vi "Main.vi"(11 "Module Admin":refnum<class "Delacor_lib_QMH_Module Admin.lvclass">) -> ()   [LabVIEW 2026, in "Replay.lvlib"]
doc: "This template is based off of the Queued Message Handler design pattern and the Queued Message Handler project template that ships with LabVIEW.\n\nThe main difference is that the queue is private to this module and communication between modules is performed via Broadcast and Request events.\n\nRequest events are wrapped in public API methods and are handled in the Event Handling Loop (EHL) of this VI. Any module can register for Broadcast events sent by this module. The EHL generates messages based on user interface actions.\n\nThe Message Handling Loop (MHL) processes messages generated by the EHL, or by other messages. The messages are string values, so new messages can be added easily to the Message Cases case structure in the MHL. Each message cluster can also provide an optional value for Message Data, which is a variant that can be converted to whatever message-specific data is required.\n_____\nBased on DQMH Dev Tools: Project Template 7.1.2.1547."
uses:
  Replay.lvlib
  <vilib>/Delacor/Delacor QMH/Libraries/Module Admin_class/Delacor_lib_QMH_Module Admin.lvclass
  <vilib>/Wovalab/Utilities/Helper Loop Periodic Timing/Late Execution Mode--enum.ctl
  <vilib>/Wovalab/Utilities/Helper Loop Periodic Timing/Helper Loop Periodic Timing.lvclass/Helper Loop Periodic Timing.ctl
  Replay MH Loop.ctl
  Replay Helper Loop.ctl
  <vilib>/Delacor/Delacor QMH/Libraries/Message Queue_class/Delacor_lib_QMH_Message Queue.lvclass/Delacor_lib_QMH_Message Queue.ctl
  Stop Argument--cluster.ctl
  <vilib>/Delacor/Delacor QMH/Libraries/Module Admin_class/Delacor_lib_QMH_Module Admin.lvclass/Delacor_lib_QMH_Module Admin.ctl
  Load UserEvents Argument--cluster.ctl
  Load UserEvents (Reply Payload)--cluster.ctl
  <vilib>/Utility/miscctls.llb/LVPointTypeDef.ctl
  modules/coordinator/src/Libraries/UserEventRecorder/KeyboardAndMouseDataAcquisition.ctl
  <vilib>/Delacor/Delacor QMH/Libraries/Message Queue_class/Delacor_lib_QMH_Enqueue Message (Single).vi
  <vilib>/Delacor/Delacor QMH/Libraries/Module Admin_class/Delacor_lib_QMH_Get External Launch.vi
  <vilib>/Wovalab/Utilities/Helper Loop Periodic Timing/Stop Helper Loop.vi
  <vilib>/Wovalab/Utilities/Helper Loop Periodic Timing/Stop Helper Loop Internal.vi
  <vilib>/Wovalab/Utilities/Helper Loop Periodic Timing/U32 Max Value--constant.vi
  <vilib>/Wovalab/Utilities/Helper Loop Periodic Timing/Update Last Execution Time.vi
  <vilib>/Wovalab/Utilities/Helper Loop Periodic Timing/Loops Events AE.vi
  <vilib>/Wovalab/Utilities/Helper Loop Periodic Timing/Notify Monitoring Window.vi
  <vilib>/Wovalab/Utilities/Helper Loop Periodic Timing/Monitoring--global.vi
  <vilib>/Wovalab/Utilities/Helper Loop Periodic Timing/Helper Loop Periodic Timing.lvclass
  <vilib>/Delacor/Delacor QMH/Libraries/Message Queue_class/Delacor_lib_QMH_Message Queue.lvclass
  modules/coordinator/src/Libraries/Launcher/Launcher.lvlib
panel:
  out "Late?":bool
  out "First Execution Since Period Modification?":bool
  out "error out":errorcluster
  out "Status":string
  in  "Simulate MHL Error":bool
  in  "Simulate EHL Error":bool
  # "Other processes communicate with this Module via its Public API (wrappers for its Request Events).\n\nThis Module communicates with other processes via its Broadcast Events.\nAny process that wants to receive these messages can register for this module's Broadcast events."
  # "This template is for the DQMH framework. See the block diagram for more information on how to use this template."
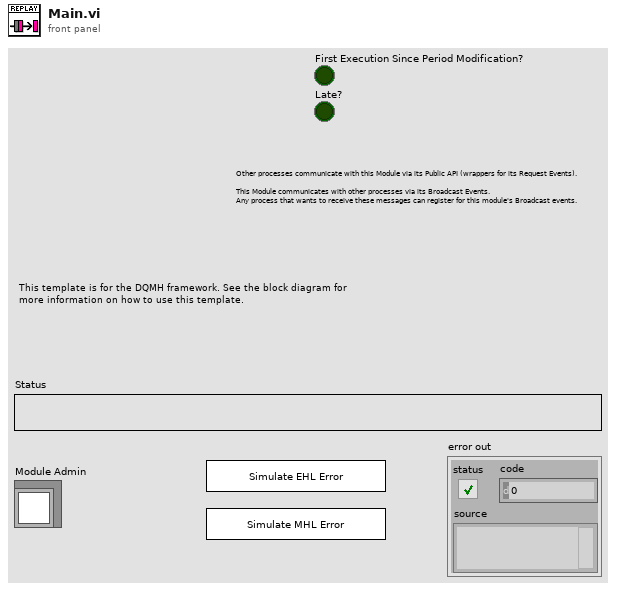
[diagram p1: front panel]
types:
  T1 = typedef "Wovalab_lib_Utilities.lvlib/Helper Loop Periodic Timing.lvclass/Late Execution Mode--enum.ctl" = enum16{"No change", "Process missed periods ignoring original phase", "Process missed periods maintaining original phase"}
  T2 = typedef "Replay.lvlib/Request Events--cluster.ctl" = cluster{"Stop Module":refnum<user-event>, "Show Panel":refnum<user-event>, "Hide Panel":refnum<user-event>, "Get Module Execution Status":refnum<user-event>, "Show Diagram":refnum<user-event>, "Set Run ID to Replay":refnum<user-event>, "Load UserEvents":refnum<user-event>, "Private.Trigger Replay Metadata":refnum<user-event>}
  T3 = typedef "Launcher.lvlib/Broadcast Events--cluster.ctl" = cluster{"Module Did Init":refnum<user-event>, "Status Updated":refnum<user-event>, "Error Reported":refnum<user-event>, "Module Did Stop":refnum<user-event>, "Update Module Execution Status":refnum<user-event>, "Start Capture Detection Loop":refnum<user-event>, "Benchmark Started":refnum<user-event>, "Broadcast number of frames and run ID":refnum<user-event>}
  T4 = typedef "Replay.lvlib/Replay Helper Loop.ctl" = cluster{"Run ID":string, "Sample Number":i32, "Load From Program Data":bool}
  T5 = typedef "Replay.lvlib/Replay MH Loop.ctl" = cluster{"Run ID":string, "Frame Index":i32}
  T6 = enum32{"invalid lock state", "Not Locked", "Locked (No Password)", "Password-protected"}
  T7 = typedef "Replay.lvlib/Stop Argument--cluster.ctl" = cluster{"Origin":string, "Exit via Stop Module Req?":bool, "Wait for Module to stop?":bool}
  T8 = typedef "Replay.lvlib/Load UserEvents Argument--cluster.ctl" = cluster{"Run ID":string, "Wait Notifier":refnum<notifier>, "wait for reply":bool, "Load From Program Data":bool}
  T9 = typedef "LVPointTypeDef.ctl" = cluster{"Horizontal":i16, "Vertical":i16}
  T10 = enum32{"Invalid", "Standard", "Closed", "Hidden", "Minimized", "Maximized"}
  T11 = typedef "Replay.lvlib/Load UserEvents (Reply Payload)--cluster.ctl" = cluster{"error":errorcluster, "Run ID":string, "Load From Program Data":bool}
  T12 = typedef "KeyboardAndMouseDataAcquisition.ctl" = cluster{"axis info":cluster{"Horizontal":i32, "Vertical":i32, "Scrolling":i32}, "button info":cluster{"button 1":bool, "button 2":bool, "button 3":bool, "button 4":bool}, "Relative Time (User Event)":dbl, "Sample Number":u32, "Relative Time (Frame 0)":dbl, "key mode":enum16{"RELATIVE", "ABSOLUTE"}, "Frame Number":u32, "Keyboard Key Pressed":enum16{"0", "1", "2", "3", "4", "5", "6", "7", "8", "9", "A", "B", "C", "D", "E", "F", "G", "H", "I", "J", "K", "L", "M", "N", "O", "P", "Q", "R", "S", "T", "U", "V", "W", "X", "Y", "Z", "F1", "F2", "F3", "F4", "F5", "F6", "F7", "F8", "F9", "F10", "F11", "F12", "F13", "F14", "F15", "ADD", "BACK", "BACKSLASH", "CAPITAL", "COMMA", "DECIMAL", "DELETE", "DIVIDE", "DOWN", "END", "EQUALS", "ESCAPE", "GRAVE (`)", "HOME", "INSERT", "LBRACKET", "LCONTROL", "LEFT", "L ALT", "LSHIFT", "LWIN", "MINUS", "MULTIPLY", "NEXT", "NUMLOCK", "NUMPAD_0", "NUMPAD_1", "NUMPAD_2", "NUMPAD_3", "NUMPAD_4", "NUMPAD_5", "NUMPAD_6", "NUMPAD_7", "NUMPAD_8", "NUMPAD_9", "PAUSE", "PERIOD", "PRIOR (PG UP)", "RBRACKET", "RCONTROL", "RETURN", "RIGHT", "R ALT", "RSHIFT", "RWIN", "SCROLL", "SEMICOLON", "SLASH", "SPACE", "SUBTRACT", "TAB", "UP", "ENTER (num pad)", "' (quote)"}, "Keyboard No Op":bool}
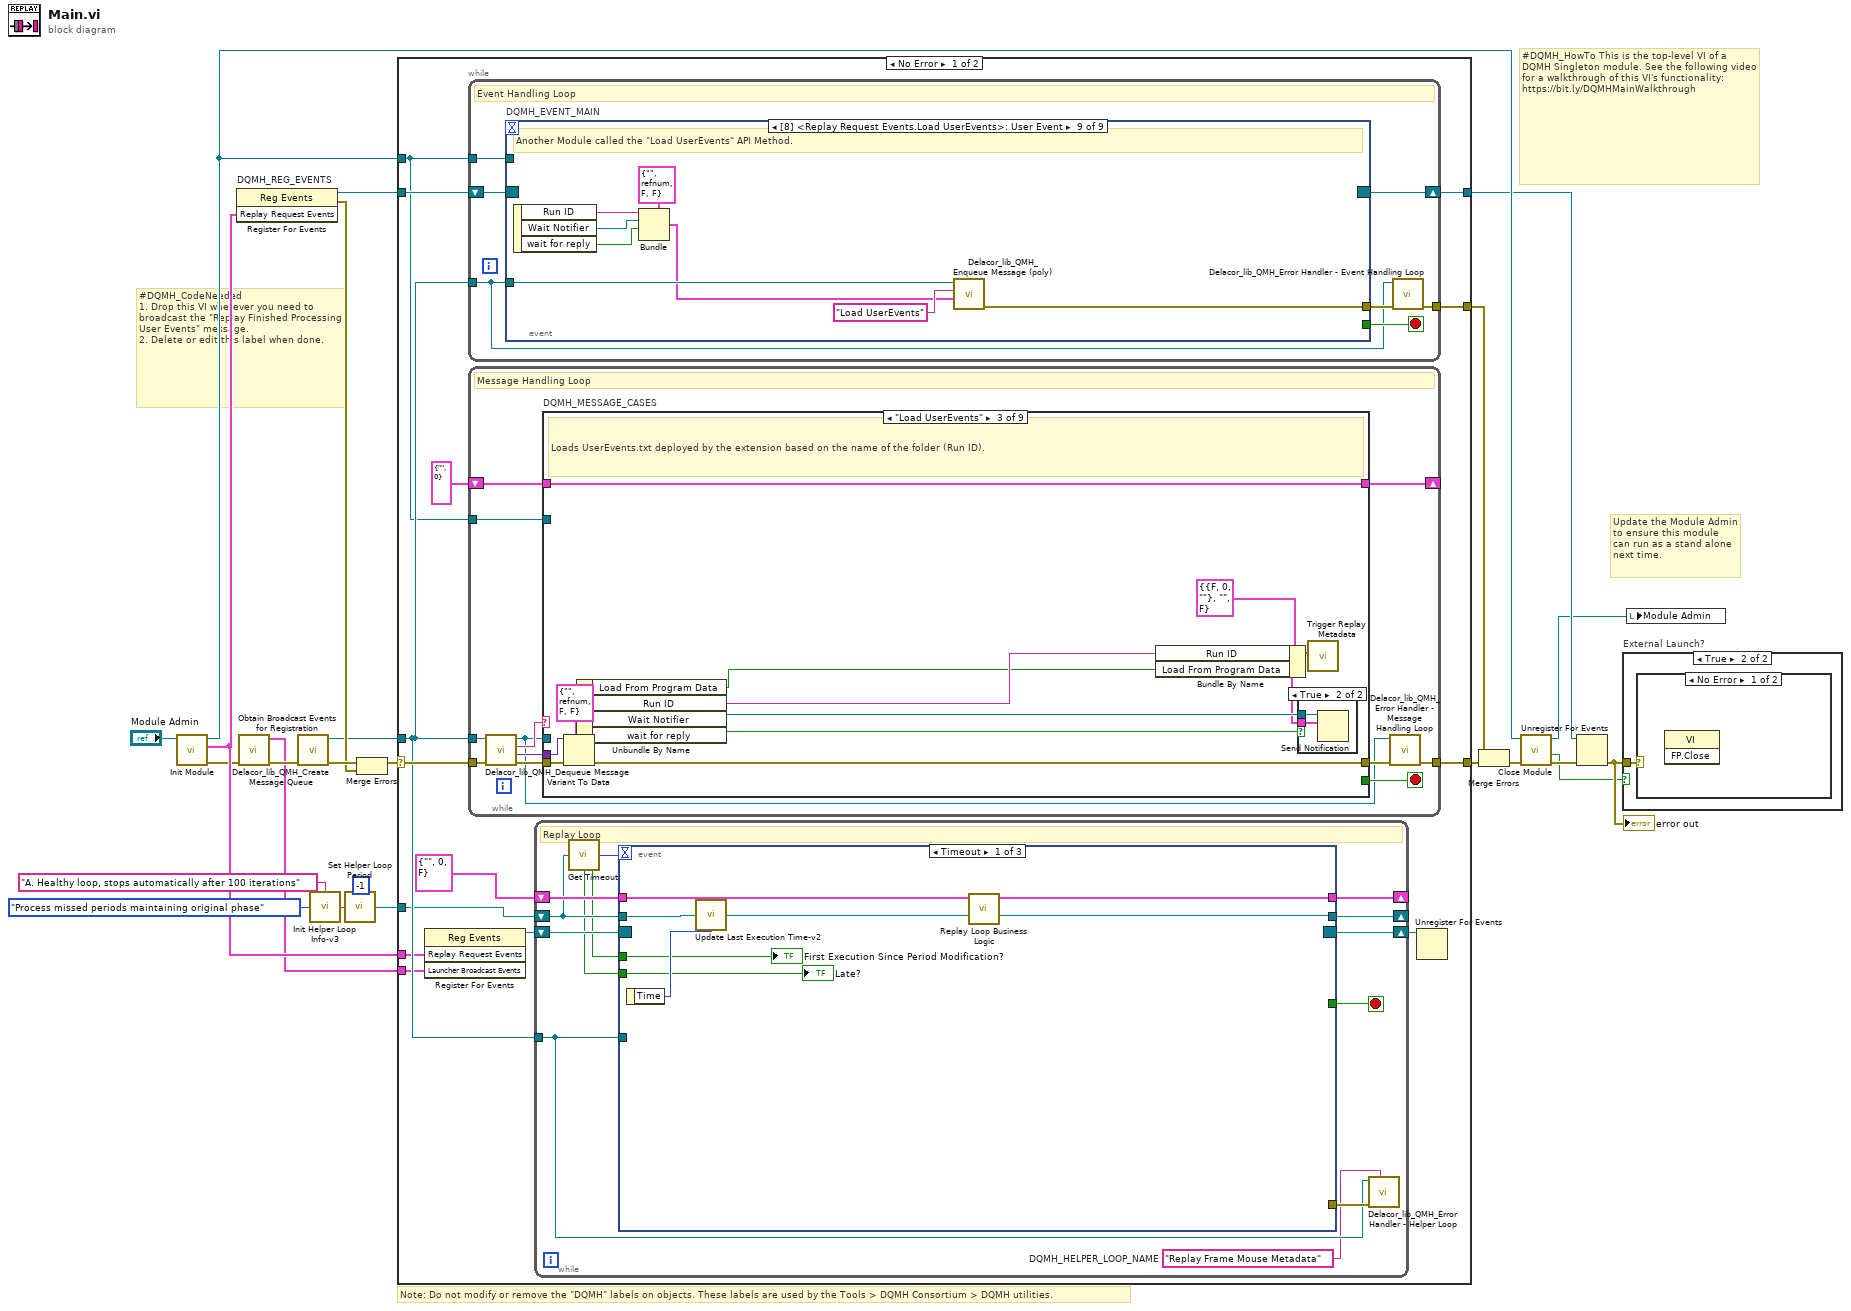
[diagram p0: block diagram]
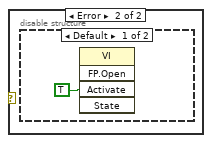
[diagram p3: hidden frame]
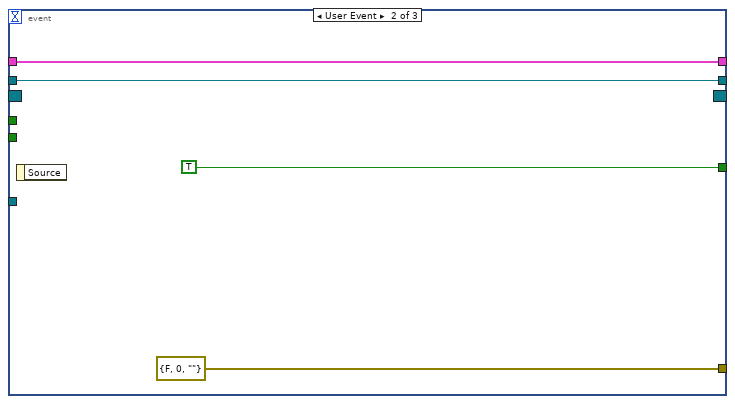
[diagram p5: hidden frame]
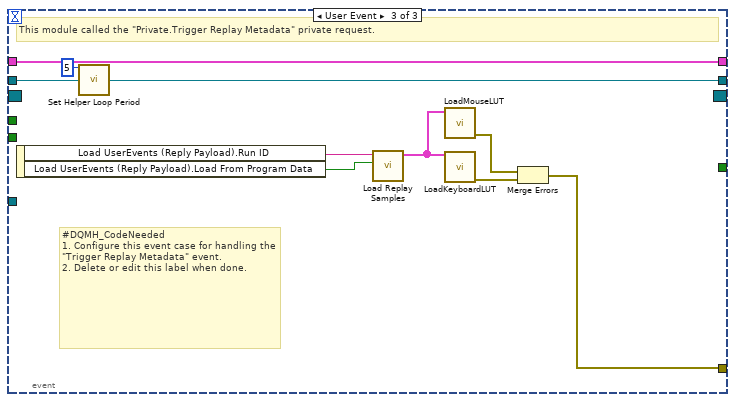
[diagram p6: hidden frame]
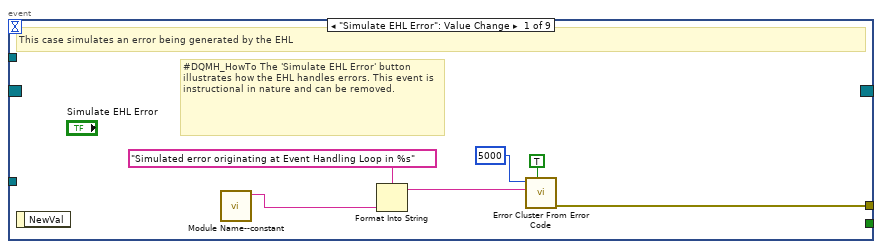
[diagram p7: hidden frame]
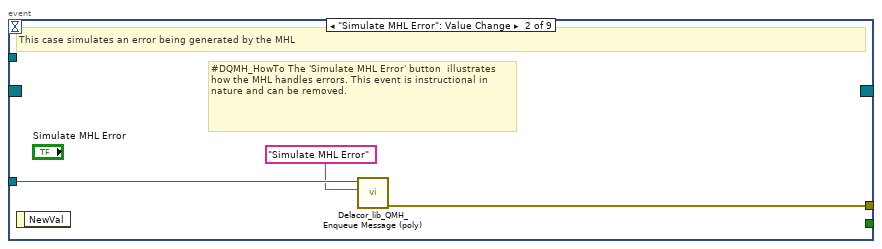
[diagram p8: hidden frame]
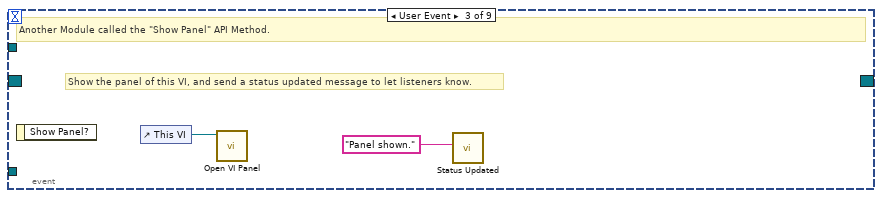
[diagram p9: hidden frame]
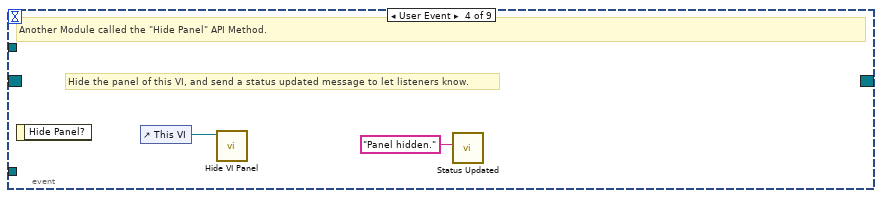
[diagram p10: hidden frame]
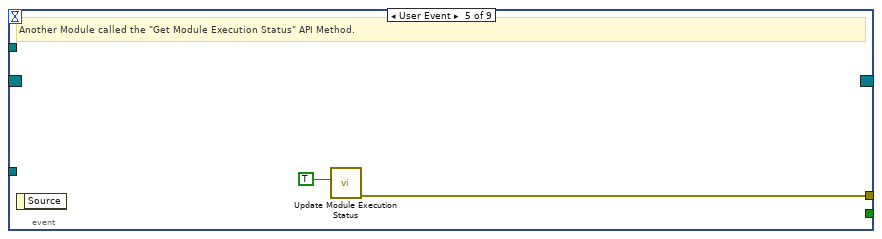
[diagram p11: hidden frame]
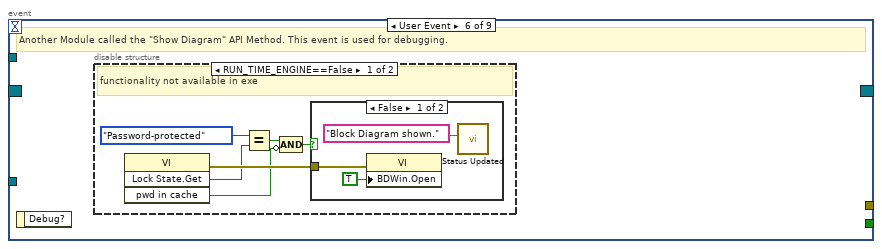
[diagram p12: hidden frame]
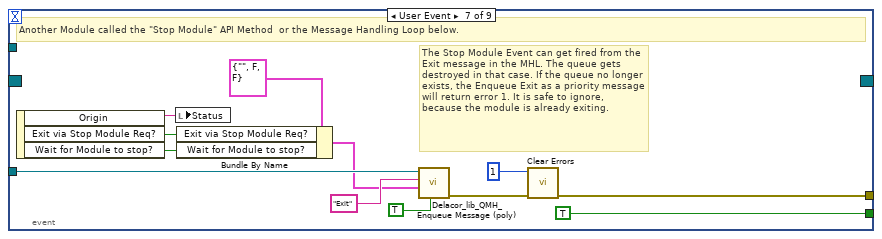
[diagram p15: hidden frame]
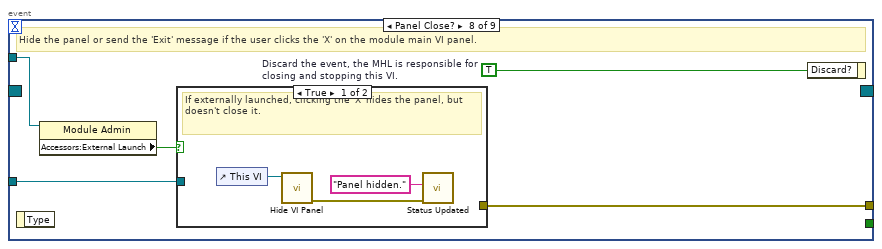
[diagram p16: hidden frame]
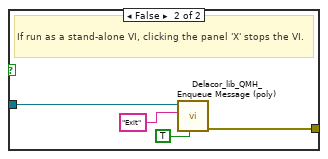
[diagram p17: hidden frame]
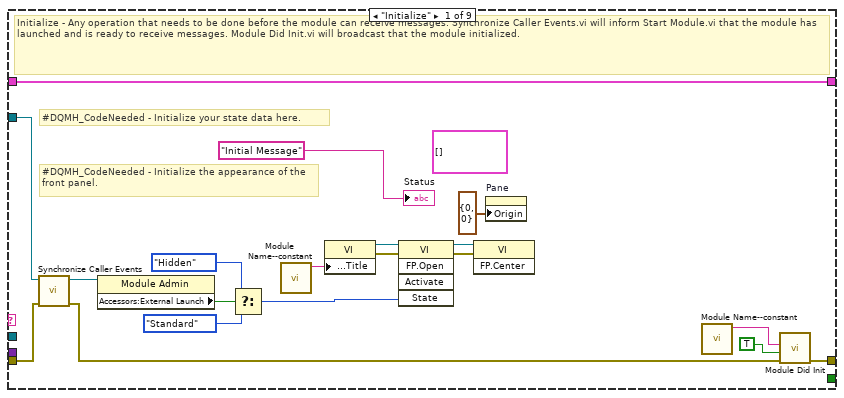
[diagram p18: hidden frame]
diagram:
  # "#DQMH_CodeNeeded\n1. Drop this VI wherever you need to fire the \"Private.Trigger Replay Metadata\" event.\n2. Delete or edit this label when done."
  # "#DQMH_CodeNeeded\n1. Drop this VI wherever you need to broadcast the \"Replay Finished Processing User Events\" message.\n2. Delete or edit this label when done."
  # "#DQMH_HowTo This is the top-level VI of a DQMH Singleton module. See the following video for a walkthrough of this VI's functionality: https://bit.ly/DQMHMainWalkthrough"
  # "Note: Do not modify or remove the \"DQMH\" labels on objects. These labels are used by the Tools > DQMH Consortium > DQMH utilities."
  # "Update the Module Admin to ensure this module can run as a stand alone next time."
  n1 = call "Init Module.vi"("Singleton Module Admin in"="Module Admin") -> ("error out"=w8:errorcluster, "Replay Request Events"=w9:T2, "Singleton Module Admin out"=w16:refnum<class "Delacor_lib_QMH_Module Admin.lvclass">)  [unwired: 8 in]
  n2 = register-events "DQMH_REG_EVENTS"(w9) -> (reference out=w14:refnum<event-registration>, error out=w17:errorcluster)  [unwired: 2 in]
  n3 = call "Obtain Broadcast Events for Registration.vi"("error in"=w8) -> ("error out"=w7:errorcluster, "Launcher Broadcast Events"=w6:T3)  [unwired: 8 in, 1 out]
  n4 = call <vilib>:"Delacor_lib_QMH_Create Message Queue.vi"("error in"=w7) -> ("error out"=w19:errorcluster, "Message Queue"=w13:refnum<class "Delacor_lib_QMH_Message Queue.lvclass">)  [unwired: 9 in]
  n5 = call <vilib>:"Init Helper Loop Info-v3.vi"("Late Execution Mode (Process missed periods ignoring original phase)"=Late_Execution_Mode--enum."Process missed periods maintaining original phase", "Loop Name (\"\": Caller VI)"="A. Healthy loop, stops automatically after 100 iterations" ("Loop Name (\"\": Caller VI)")) -> ("Helper Loop Periodic Timing"=w4:refnum<class "Helper Loop Periodic Timing.lvclass">)
  n6 = call <vilib>:"Set Helper Loop Period.vi"("Period (ms)"=-1, "Helper Loop Periodic Timing in"=w4) -> ("Helper Loop Periodic Timing out"=w2:refnum<class "Helper Loop Periodic Timing.lvclass">)  [unwired: 13 in]
  n7 = Merge Errors(w19, w17) -> (w18:errorcluster)
  n8 = case shown="No Error" w18 {
    selector: w18 -> [w36 w246]
    tunnel: [w38 w245] -> w24
    tunnel: [w35 w244] -> w15
    tunnel: w14 -> [w34 w244]
    tunnel: w13 -> [w33 w239]
    tunnel: [w37 _] -> w22
    tunnel: w16 -> [w32 w240]
    tunnel: w9 -> [w31 _]
    tunnel: w6 -> [w28 _]
    tunnel: w2 -> [w27 _]
    frame No Error {
      n9 = register-events ("DQMH_HELPER_REGFOREVENTS")(w31, w28) -> (reference out=w29:refnum<event-registration>)  [unwired: 2 in, 1 out]
      n10 = while {
        tunnel: w33 -> [w73]
        shift-right: [w76] -> w35
        shift-left: w34 -> [w77]
        tunnel: [w78] -> w37
        tunnel: w32 -> [w74]
        stop <- w75 stop-if-true
        # "Event Handling Loop"
        n11 = event "DQMH_EVENT_MAIN" shown="[8] <Replay Request Events.Load UserEvents>: User Event" {
          selector: w77 -> [_ _ _ _ _ _ _ _ _]
          dyn-events: [_ _ _ _ _ _ _ _ _] -> w76
          timeout: _ -> [_ _ _ _ _ _ _ _ _]
          tunnel: [_ _ _ _ _ _ TRUE ("Discard?") _ _] -> w75
          tunnel: w73 -> [_ w87 _ _ _ _ w111 w118 w135]
          tunnel: [w85 w88 _ _ w94 _ w114 w120 w128] -> w79
          tunnel: w74 -> [_ _ _ _ _ _ _ w117 _]
          event "Simulate EHL Error": Value Change {
            # "#DQMH_HowTo The 'Simulate EHL Error' button  illustrates how the EHL handles errors. This event is instructional in nature and can be removed."
            # "This case simulates an error being generated by the EHL"
            n12 = event-data() -> ()  [unwired: 1 in, 1 out]
            n13 = call "Module Name--constant.vi"() -> ("Module Name"=w82:string)  [unwired: 11 in]
            n14 = Format Into String(format string="Simulated error originating at Event Handling Loop in %s", w82) -> (resulting string=w83:string)  [unwired: 2 in, 1 out]
            n15 = call <vilib>:"Error Cluster From Error Code.vi"("show call chain? (False)"=TRUE, "error message (\"\")"=w83, "error code (0)"=5000) -> ("error out"=w85:errorcluster)  [unwired: 6 in]
          }
          event "Simulate MHL Error": Value Change {
            # "#DQMH_HowTo The 'Simulate MHL Error' button  illustrates how the MHL handles errors. This event is instructional in nature and can be removed."
            # "This case simulates an error being generated by the MHL"
            n16 = event-data() -> ()  [unwired: 1 in, 1 out]
            n17 = call-poly <vilib>:"Delacor_lib_QMH_Enqueue Message (poly).vi"("Message"="Simulate MHL Error", "Message Queue in"=w87) -> ("error out"=w88:errorcluster)  [unwired: 8 in, 1 out]
          }
          event User Event {
            # "Show the panel of this VI, and send a status updated message to let listeners know."
            # "Another Module called the \"Show Panel\" API Method."
            n18 = event-data() -> ()  [unwired: 1 in, 1 out]
            n19 = control-ref of="This VI"() -> (w90:refnum<vi>)
            n20 = call "Open VI Panel.vi"("VI"=w90) -> ()  [unwired: 10 in, 1 out]
            n21 = call "Status Updated.vi"("Status"="Panel shown." ("format string")) -> ()  [unwired: 10 in, 1 out]
          }
          event User Event {
            # "Hide the panel of this VI, and send a status updated message to let listeners know."
            # "Another Module called the \"Hide Panel\" API Method."
            n22 = event-data() -> ()  [unwired: 1 in, 1 out]
            n23 = control-ref of="This VI"() -> (w92:refnum<vi>)
            n24 = call "Hide VI Panel.vi"("VI"=w92) -> ()  [unwired: 10 in, 1 out]
            n25 = call "Status Updated.vi"("Status"="Panel hidden." ("format string")) -> ()  [unwired: 10 in, 1 out]
          }
          event User Event {
            # "Another Module called the \"Get Module Execution Status\" API Method."
            n26 = event-data() -> ()  [unwired: 1 in, 1 out]
            n27 = call "Update Module Execution Status.vi"("Running?"=TRUE) -> ("error out"=w94:errorcluster)  [unwired: 10 in]
          }
          event User Event {
            # "Another Module called the \"Show Diagram\" API Method. This event is used for debugging."
            n28 = event-data() -> ()  [unwired: 1 in, 1 out]
            n29 = disable-structure shown="RUN_TIME_ENGINE==False" {
              frame condition #0 (active) {
                # "functionality not available in exe"
                n30 = invoke on="Invoke Node" class="VI" method="Lock State.Get"() -> (error out=w100:errorcluster, "Get Lock State"=w99:T6, "pwd in cache"=w96:bool)  [unwired: 4 in, 1 out]
                n31 = Equal?(x=T6."Password-protected", y=w99) -> (x = y?=w97:bool)
                n32 = Compound Arithmetic op=AND(w97, invert w96) -> (w95:bool)
                n33 = case shown="False" w95 {
                  tunnel: w100 -> [w103 _]
                  frame False {
                    n34 = property on="Property Node" class="VI"(error in=w103, "BDWin.Open"=TRUE ("Block Diagram Window:Open")) -> ()  [unwired: 1 in, 2 out]
                    n35 = call "Status Updated.vi"("Status"="Block Diagram shown." ("format string")) -> ()  [unwired: 10 in, 1 out]
                  }
                  frame True {
                    # "Password-protected VI, and the password is not in the cache. Do not show the diagram."
                  }
                }
              }
              frame condition #1 {
              }
            }
          }
          event User Event {
            # "The Stop Module Event can get fired from the Exit message in the MHL. The queue gets destroyed in that case. If the queue no longer exists, the Enqueue Exit as a priority message will return error 1. It is safe to ignore, because the module is already exiting."
            # "Another Module called the \"Stop Module\" API Method  or the Message Handling Loop below."
            n36 = event-data() -> ("Origin"=w110:string, "Exit via Stop Module Req?"=w106:bool, "Wait for Module to stop?"=w105:bool)  [unwired: 1 in]
            n37 = local write "Status"(w110) -> ()
            n38 = Bundle By Name(cluster=T7 {"Origin"="", "Exit via Stop Module Req?"=FALSE, "Wait for Module to stop?"=FALSE} ("Stop Argument"), "Exit via Stop Module Req?"=w106, "Wait for Module to stop?"=w105) -> (w104:T7)
            n39 = call-poly <vilib>:"Delacor_lib_QMH_Enqueue Message (poly).vi"("Priority Message? (F)"=TRUE, "Message Data"=w104, "Message"="Exit", "Message Queue in"=w111) -> ("error out"=w115:errorcluster)  [unwired: 6 in, 1 out]
            n40 = call <vilib>:"Clear Errors.vi"("error in (no error)"=w115, "specific error code to clear (0: all)"=1) -> ("error out"=w114:errorcluster)  [unwired: 4 in, 1 out]
          }
          event Panel Close? {
            w119 = TRUE  # Discard the event, the MHL is responsible for closing and stopping this VI.
            # "Hide the panel or send the 'Exit' message if the user clicks the 'X' on the module main VI panel."
            n41 = event-data() -> ()  [unwired: 1 in, 1 out]
            n42 = property on="Property Node" class="Module Admin"(reference=w117) -> ("Accessors:External Launch"=w116:bool)  [unwired: 1 in, 2 out]
            n43 = case shown="True" w116 {
              tunnel: w118 -> [_ w126]
              tunnel: [_ w127] -> w120
              frame True {
                # "If externally launched, clicking the 'X' hides the panel, but doesn't close it."
                n44 = control-ref of="This VI"() -> (w123:refnum<vi>)
                n45 = call "Hide VI Panel.vi"("VI"=w123) -> ("error out"=w121:errorcluster)  [unwired: 10 in]
                n46 = call "Status Updated.vi"("error in"=w121, "Status"="Panel hidden." ("format string")) -> ()  [unwired: 9 in, 1 out]
              }
              frame False {
                # "If run as a stand-alone VI, clicking the panel 'X' stops the VI."
                n47 = call-poly <vilib>:"Delacor_lib_QMH_Enqueue Message (poly).vi"("Priority Message? (F)"=TRUE, "Message"="Exit", "Message Queue in"=w126) -> ("error out"=w127:errorcluster)  [unwired: 7 in, 1 out]
              }
            }
            n48 = event-data ("Event Filter Node")("Discard?"=w119) -> ()  [unwired: 1 in, 1 out]
          }
          event User Event {
            # "Another Module called the \"Load UserEvents\" API Method."
            n49 = event-data() -> ("Run ID"=w131:string, "Wait Notifier"=w130:refnum<notifier>, "wait for reply"=w129:bool)  [unwired: 1 in]
            n50 = Bundle(cluster=T8 {"Run ID"="", "Wait Notifier"=refnum, "wait for reply"=FALSE, "Load From Program Data"=FALSE} ("Load UserEvents Argument"), "Run ID"=w131, "Wait Notifier"=w130, "wait for reply"=w129) -> (w132:T8)  [unwired: 1 in]
            n51 = call-poly <vilib>:"Delacor_lib_QMH_Enqueue Message (poly).vi"("Message Data"=w132, "Message"="Load UserEvents", "Message Queue in"=w135) -> ("error out"=w128:errorcluster)  [unwired: 7 in, 1 out]
          }
        }
        n52 = call-dynamic "Delacor_lib_QMH_Error Handler - Event Handling Loop.vi"("error in"=w79, "Message Queue in"=w73) -> ("dup error in"=w78:errorcluster)  [unwired: 8 in, 1 out]
      }
      n53 = while {
        tunnel: w33 -> [w136]
        shift-right: [w144] -> _
        shift-left: T5 {"Run ID"="", "Frame Index"=0} ("Replay MH Loop") -> [w145]
        tunnel: w36 -> [w147]
        tunnel: [w139] -> w38
        tunnel: w32 -> [w140]
        stop <- w143 stop-if-true
        # "Message Handling Loop"
        n54 = call-dynamic "Delacor_lib_QMH_Dequeue Message.vi"("error in"=w147, "Message Queue in"=w136) -> ("error out"=w146:errorcluster, "Message Data"=w141:variant, "Message"=w142:string, "Message Queue out"=w137:refnum<class "Delacor_lib_QMH_Message Queue.lvclass">)  [unwired: 6 in]
        n55 = case "DQMH_MESSAGE_CASES" shown="\"Load UserEvents\"" w142 {
          selector: w142 -> [_ _ _ _ _ _ _ _ w234]
          tunnel: w137 -> [_ _ _ _ _ _ w200 w222 _]
          tunnel: w146 -> [w164 w168 w180 w185 w187 w196 w207 w228 w237]
          tunnel: [w162 w168 w179 w184 w187 w195 w203 w223 w238] -> w138
          tunnel: w145 -> [w148 w167 w171 w183 w186 w193 w202 w221 w235]
          tunnel: [w148 w167 w171 w183 w186 w193 w202 w221 w235] -> w144
          tunnel: [_ _ _ _ _ _ _ w220 _] -> w143
          tunnel: w141 -> [_ _ w178 _ _ _ w201 w219 _]
          tunnel: w140 -> [w154 _ _ _ _ _ w199 w214 _]
          frame "Initialize" {
            (unwired) T12[] [] ("Array")
            # "#DQMH_CodeNeeded - Initialize the appearance of the front panel."
            # "#DQMH_CodeNeeded - Initialize your state data here."
            # "Initialize - Any operation that needs to be done before the module can receive messages. Synchronize Caller Events.vi will inform Start Module.vi that the module has launched and is ready to receive messages. Module Did Init.vi will broadcast that the module initialized."
            n56 = call "Synchronize Caller Events.vi"("error in"=w164, "Singleton Module Admin in"=w154) -> ("error out"=w163:errorcluster, "Singleton Module Admin out"=w151:refnum<class "Delacor_lib_QMH_Module Admin.lvclass">)  [unwired: 8 in]
            n57 = property on="Property Node" class="Module Admin"(reference=w151) -> ("Accessors:External Launch"=w158:bool)  [unwired: 1 in, 2 out]
            n58 = Select(t=T10."Hidden" ("State"), s=w158, f=T10."Standard" ("State")) -> (s? t:f=w155:T10)
            n59 = call "Module Name--constant.vi"() -> ("Module Name"=w161:string)  [unwired: 11 in]
            n60 = property on="Property Node" class="VI"("Front Panel.Title"=w161) -> (reference out=w160:refnum<vi>, error out=w166:errorcluster)  [unwired: 2 in]
            n61 = invoke on="Invoke Node" class="VI" method="FP.Open"(reference=w160, error in=w166, "State"=w155) -> (reference out=w159:refnum<vi>, error out=w165:errorcluster)  [unwired: 2 in, 3 out]
            n62 = invoke on="Invoke Node" class="VI" method="FP.Center"(reference=w159, error in=w165) -> ()  [unwired: 1 in, 3 out]
            n63 = property on="Pane" class="Pane"("Origin"=T9 {"Horizontal"=0, "Vertical"=0}) -> ()  [unwired: 2 in, 2 out]
            n64 = call "Module Name--constant.vi"() -> ("Module Name"=w152:string)  [unwired: 11 in]
            n65 = call "Module Did Init.vi"("error in"=w163, "Initialized?"=TRUE, "Origin"=w152) -> ("error out"=w162:errorcluster)  [unwired: 8 in]
            "Status" <- "Initial Message" ("Initial Message")
          }
          frame "---Module Specific---" {
            # "Separator -- The following cases handle messages specific to this Module."
          }
          frame "Load UserEvents" {
            # "Loads UserEvents.txt deployed by the extension based on the name of the folder (Run ID)."
            n66 = Variant To Data(error in=w180, type=T8 {"Run ID"="", "Wait Notifier"=refnum, "wait for reply"=FALSE, "Load From Program Data"=FALSE} ("Load UserEvents Argument"), Variant=w178) -> (data=w176:T8, error out=w179:errorcluster)
            n67 = Unbundle By Name(w176) -> ("Load From Program Data"=w169:bool, "Run ID"=w170:string, "Wait Notifier"=w175:refnum<notifier>, "wait for reply"=w174:bool)
            n68 = Bundle By Name(cluster=T11 {"error"={"status"=FALSE, "code"=0, "source"=""}, "Run ID"="", "Load From Program Data"=FALSE} ("Load UserEvents (Reply Payload)"), "Run ID"=w170, "Load From Program Data"=w169) -> (w172:T11)
            n69 = case "DQMH_FIRE_NOTIFIER" shown="True" w174 {
              tunnel: w175 -> [_ w182]
              tunnel: w172 -> [_ w181]
              frame False {
              }
              frame True {
                n70 = Send Notification(notification=w181, notifier=w182) -> ()  [unwired: 1 in, 2 out]
              }
            }
            n71 = call "Trigger Replay Metadata.vi"("Load UserEvents (Reply Payload)"=w172) -> ()  [unwired: 10 in, 1 out]
          }
          frame "---Copy This Frame---" {
            # "Duplicate this frame when creating new messages.  Change this comment in the duplicated frame to describe this message."
            n72 = Merge Errors(w185) -> (w184:errorcluster)
          }
          frame "---Exit and Error Handling---" {
            # "Separator - The following cases handle errors and exit messages."
          }
          frame "Simulate MHL Error" {
            # "#DQMH_HowTo The 'Simulate MHL Error' button  illustrates how the MHL handles errors. This event is instructional in nature and can be removed."
            # "Simulate an error occurring at the MHL"
            n73 = call "Module Name--constant.vi"() -> ("Module Name"=w189:string)  [unwired: 11 in]
            n74 = Format Into String(format string="Simulated error originating at Message Handling Loop in %s", w189) -> (resulting string=w190:string)  [unwired: 2 in, 1 out]
            n75 = call <vilib>:"Error Cluster From Error Code.vi"("show call chain? (False)"=TRUE, "error message (\"\")"=w190, "error code (0)"=5001) -> ("error out"=w194:errorcluster)  [unwired: 6 in]
            n76 = Merge Errors(w196, w194) -> (w195:errorcluster)
          }
          frame "Error" {
            # "#DQMH_CodeRecommended - If the module is running in standalone mode (External Launch = FALSE), this code will pop up an error dialog and call the 'Exit' message if an error occurs. Add more fine-grained error management here."
            # "Error - Check the error message data and respond accordingly. This message is sent by the \"Error Handler\" VIs at the end of each loop in this application."
            n77 = property on="Property Node" class="Module Admin"(reference=w199) -> ("Accessors:External Launch"=w198:bool)  [unwired: 1 in, 2 out]
            n78 = Variant To Data(error in=w207, type=errorcluster {"status"=FALSE, "code"=0, "source"=""} ("error constant"), Variant=w201) -> (data=w197:errorcluster, error out=w205:errorcluster)
            n79 = local write "error out"(w197) -> ()
            n80 = call "Error Reported.vi"("Error"=w197) -> ()  [unwired: 10 in, 1 out]
            n81 = case shown="False" w198 {
              tunnel: [w212 _] -> w204
              tunnel: w200 -> [w210 _]
              tunnel: w197 -> [w211 _]
              frame False {
                n82 = disable-structure shown="Default" {
                  disable-tunnel: w211 -> [w213 _]
                  frame condition #0 (active) {
                    # "If the module is running standalone, then pop up an error dialog and call the \"Exit\" message."
                    n83 = call <vilib>:"Simple Error Handler.vi"("error in (no error)"=w213) -> ()  [unwired: 4 in, 5 out]
                  }
                  frame condition #1 {
                    # "To prevent the Simple Error Handler VI from being loaded (e.g. when deploying to a Real-Time target), add the Conditional Disable Symbol \"DQMH_Disable_SEH\" to your project and set it to TRUE."
                  }
                }
                n84 = call-poly <vilib>:"Delacor_lib_QMH_Enqueue Message (poly).vi"("Priority Message? (F)"=TRUE, "Message"="Exit", "Message Queue in"=w210) -> ("error out"=w212:errorcluster)  [unwired: 7 in, 1 out]
              }
              frame True {
                # "If the module was launched externally, calling the Error Reported broadcast VI is the only action performed by the \"Error\" message. The module's caller can then process the error appropriately."
              }
            }
            n85 = Merge Errors(w205, w204) -> (w203:errorcluster)
          }
          frame "Exit" {
            w218 = 91  # 91: not all Exit messages will have an argument
            w220 = TRUE  # Stop the VI
            # "Release the message queue reference"
            # "#DQMH_CodeNeeded - Add any required cleanup code here."
            # "Exit - Exit the application."
            n86 = Variant To Data(error in=w228, type=T7 {"Origin"="", "Exit via Stop Module Req?"=FALSE, "Wait for Module to stop?"=FALSE} ("Stop Argument"), Variant=w219) -> (data=w216:T7, error out=w225:errorcluster)
            n87 = call <vilib>:"Clear Errors.vi"("error in (no error)"=w225, "specific error code to clear (0: all)"=w218) -> ("error out"=w227:errorcluster)  [unwired: 4 in, 1 out]
            n88 = control-ref of="This VI"() -> (w215:refnum<vi>)
            n89 = call-dynamic "Delacor_lib_QMH_Release Message Queue.vi"("error in"=w227, "Message Queue"=w222) -> ("error out"=w226:errorcluster)  [unwired: 9 in]
            n90 = call "Handle Exit.vi"("Stop Argument"=w216, "Admin in"=w214, "VI reference"=w215) -> ("error out"=w224:errorcluster)  [unwired: 7 in, 1 out]
            n91 = Merge Errors(w226, w224) -> (w223:errorcluster)
            n92 = call "Error Reported.vi"("Error"=w223) -> ()  [unwired: 10 in, 1 out]
          }
          frame Default {
            # "'Default' case only runs if there is a message that isn't defined in any of the other cases.  Output a programming error."
            n93 = call "Module Name--constant.vi"() -> ("Module Name"=w233:string)  [unwired: 11 in]
            n94 = Format Into String(format string="The invalid message string \"%s\" was received in the Message Handling Loop for module \"%s\".", w234, w233) -> (resulting string=w229:string)  [unwired: 2 in, 1 out]
            n95 = call <vilib>:"Error Cluster From Error Code.vi"("show call chain? (False)"=TRUE, "error message (\"\")"=w229, "error code (0)"=1) -> ("error out"=w236:errorcluster)  [unwired: 6 in]
            n96 = Merge Errors(w237, w236) -> (w238:errorcluster)
          }
        }
        n97 = call-dynamic "Delacor_lib_QMH_Error Handler - Message Handling Loop.vi"("error in"=w138, "Message Queue in"=w137) -> ("dup error in"=w139:errorcluster)  [unwired: 8 in, 1 out]
      }
      n98 = while "DQMH_HELPER_LOOP" {
        shift-right: [w51] -> _
        shift-left: T4 {"Run ID"="", "Sample Number"=0, "Load From Program Data"=FALSE} ("Replay MH Loop") -> [w44]
        shift-right: [w49] -> w30
        shift-left: w29 -> [w50]
        tunnel: w33 -> [w46]
        shift-right: [w41] -> _
        shift-left: w27 -> [w42]
        stop <- w48 stop-if-true
        w45 = "Replay Frame Mouse Metadata"  # DQMH_HELPER_LOOP_NAME
        # "Replay Loop"
        n99 = call <vilib>:"Get Timeout.vi"("Helper Loop Periodic Timing"=w42) -> ("Timeout (ms)"=w43:i32, "Late?"=w39:bool, "First Execution Since Period Modification?"=w40:bool)  [unwired: 12 in]
        n100 = event "DQMH_HELPER_EVENT_STRUCTURE" shown="[0] Timeout" {
          selector: w50 -> [_ _ _]
          dyn-events: [_ _ _] -> w49
          timeout: w43 -> [_ _ _]
          tunnel: w44 -> [w53 w62 w69]
          tunnel: [w52 w62 w69] -> w51
          tunnel: [_ TRUE _] -> w48
          tunnel: [_ errorcluster {"status"=FALSE, "code"=0, "source"=""} ("error constant") w65] -> w47
          tunnel: w46 -> [_ _ _]
          tunnel: w42 -> [w58 w59 w72]
          tunnel: [w57 w59 w71] -> w41
          tunnel: w40 -> [w55 _ _]
          tunnel: w39 -> [w54 _ _]
          event Timeout {
            n101 = event-data() -> ("Time"=w56:u32)  [unwired: 1 in]
            n102 = call <vilib>:"Update Last Execution Time-v2.vi"("Time"=w56, "Helper Loop Periodic Timing in"=w58) -> ("Helper Loop Periodic Timing out"=w57:refnum<class "Helper Loop Periodic Timing.lvclass">)  [unwired: 12 in, 1 out]
            n103 = call "Replay Loop Business Logic.vi"("Replay Helper Loop In"=w53) -> ("Replay Helper Loop Out"=w52:T4)  [unwired: 10 in]
            "First Execution Since Period Modification?" <- w55
            "Late?" <- w54
          }
          event User Event {
            n104 = event-data() -> ()  [unwired: 1 in, 1 out]
          }
          event User Event {
            # "#DQMH_CodeNeeded\n1. Configure this event case for handling the \"Trigger Replay Metadata\" event.\n2. Delete or edit this label when done."
            # "This module called the \"Private.Trigger Replay Metadata\" private request."
            n105 = event-data() -> ("Load UserEvents (Reply Payload).Run ID"=w68:string, "Load UserEvents (Reply Payload).Load From Program Data"=w63:bool)  [unwired: 1 in]
            n106 = call <vilib>:"Set Helper Loop Period.vi"("Period (ms)"=5, "Helper Loop Periodic Timing in"=w72) -> ("Helper Loop Periodic Timing out"=w71:refnum<class "Helper Loop Periodic Timing.lvclass">)  [unwired: 13 in]
            n107 = call "Load Replay Samples.vi"("Load From ProgramData"=w63, "Run ID"=w68) -> ("ReplaySamples"=w67:T12[])  [unwired: 8 in, 1 out]
            n108 = call "LoadMouseLUT.vi"("Metadata"=w67) -> ("error out"=w66:errorcluster)  [unwired: 10 in]
            n109 = call "LoadKeyboardLUT.vi"("Metadata"=w67) -> ("error out"=w64:errorcluster)  [unwired: 9 in, 1 out]
            n110 = Merge Errors(w66, w64) -> (w65:errorcluster)
          }
        }
        n111 = call-dynamic "Delacor_lib_QMH_Error Handler - Helper Loop.vi"("Error Debug"=w45, "error in"=w47, "Message Queue in"=w46) -> ()  [unwired: 7 in, 2 out]
      }
      n112 = Unregister For Events(event registration refnum=w30) -> ()  [unwired: 1 in, 1 out]
    }
    frame Error {
      # "Synchronize Caller Events.vi will inform Start Module.vi that the module has launched and will let the code calling Start Module.vi register for broadcasts and would permit the caller receive the broadcast that an error occurred at launch time."
      n113 = call-dynamic "Delacor_lib_QMH_Release Message Queue.vi"("error in"=w246, "Message Queue"=w239) -> ("error out"=w245:errorcluster)  [unwired: 9 in]
      n114 = call "Synchronize Caller Events.vi"("Singleton Module Admin in"=w240) -> ("error out"=w247:errorcluster)  [unwired: 9 in, 1 out]
      n115 = call "Module Name--constant.vi"() -> ("Module Name"=w243:string)  [unwired: 11 in]
      n116 = Format Into String(format string="An error occurred during initialization. %s is no longer running.", w243) -> (resulting string=w241:string)  [unwired: 2 in, 1 out]
      n117 = Merge Errors(w245, w247) -> (w248:errorcluster)
      n118 = call "Error Reported.vi"("Additional Information"=w241, "Error"=w248) -> ()  [unwired: 9 in, 1 out]
    }
  }
  n119 = Merge Errors(w22, w24) -> (w21:errorcluster)
  n120 = call "Close Module.vi"("error in"=w21, "Module Admin in"=w16) -> ("error out"=w23:errorcluster, "External Launch"=w10:bool, "Module Admin out"=w11:refnum<class "Delacor_lib_QMH_Module Admin.lvclass">)  [unwired: 7 in]
  n121 = Unregister For Events(event registration refnum=w15, error in=w23) -> (error out=w20:errorcluster)
  "error out" <- w20
  n122 = case "External Launch?" shown="True" w10 {
    tunnel: w20 -> [_ w249]
    frame False {
    }
    frame True {
      n123 = case shown="No Error" w249 {
        frame No Error {
          n124 = invoke on="Invoke Node" class="VI" method="FP.Close"() -> ()  [unwired: 3 in, 3 out]
        }
        frame Error {
          n125 = disable-structure shown="Default" {
            frame condition #0 (active) {
              n126 = invoke class="VI" method="FP.Open"("Activate"=TRUE ("Activate?")) -> ()  [unwired: 4 in, 5 out]
            }
            frame condition #1 {
              # "Don't show panel on error if running inside a built EXE."
            }
          }
        }
      }
    }
  }
  n127 = local write "Module Admin"(w11) -> ()
